vi "Display n or dt.vi"(8 "error in (no error)":errorcluster, 10 "X Scale":enum16{"time", "samples"}(ring) caption="Enum 3", 11 "Input Waveforms":waveform(dbl)[](array[waveform])) -> (0 "error out":errorcluster, 3 "Output Waveforms":waveform(dbl)[](array[waveform]))   [LabVIEW 2019, in "Instrument.Lockin.lvlib" / "Instrument UI.Lockin.lvclass"]
uses:
  Instrument UI.Lockin.lvclass
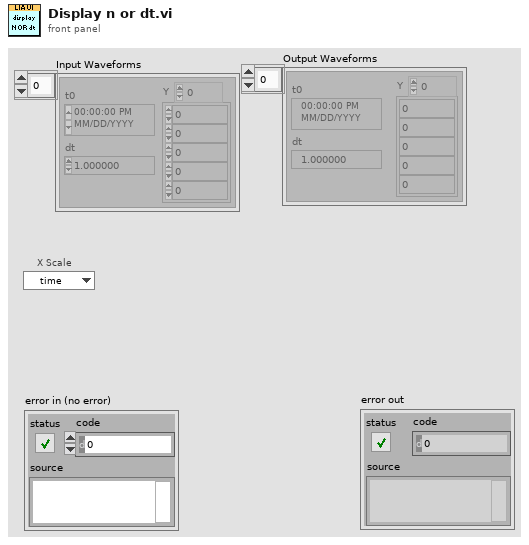
[diagram p1: front panel]
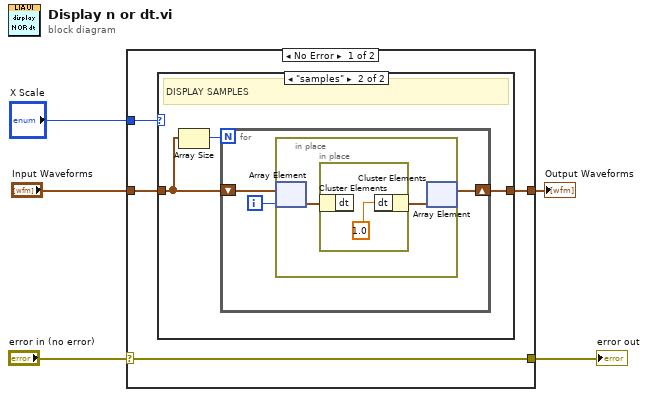
[diagram p0: block diagram]
diagram:
  n1 = case shown="No Error" "error in (no error)" {
    selector: "error in (no error)" -> [w7 w21]
    tunnel: [w9 w20] -> w5
    tunnel: "Input Waveforms" -> [w8 w20]
    tunnel: [w7 w21] -> w2
    tunnel: "X Scale" -> [w6 _]
    frame No Error {
      n2 = case shown="\"samples\"" w6 {
        tunnel: [w10 w13] -> w9
        tunnel: w8 -> [w10 w11]
        frame "time", Default {
          # "Display Time"
        }
        frame "samples" {
          # "DISPLAY SAMPLES"
          n3 = Array Size(array=w11) -> (size(s)=w12:i32)
          n4 = for {
            N: w12 -> [_]
            shift-right: [w14] -> w13
            shift-left: w11 -> [w15]
            i -> [w16]
            n5 = in-place {
              n6 = in-place-array #1(w15, w16) -> (w18:waveform(dbl))
              n7 = in-place {
                n8 = in-place-cluster #2(w18) -> ()  [unwired: 1 out]
                n9 = in-place-cluster #2("dt"=1.0) -> (w17:waveform(dbl))
              }
              n10 = in-place-array #1(w17) -> (w14:waveform(dbl)[])  [unwired: 1 out]
            }
          }
        }
      }
    }
    frame Error {
    }
  }
  "Output Waveforms" <- w5
  "error out" <- w2
